vi "Create My API.vi"(5 "My API in":refnum<class "My API.lvclass">, 8 "error in (no error)":errorcluster) -> (0 "error out":errorcluster, 3 "My API out":refnum<class "My API.lvclass">)   [LabVIEW 2017, in "My API.lvclass"]
uses:
  My API.lvclass
  My API.lvclass/My API.ctl
  classes/REST Client/REST Client.lvclass
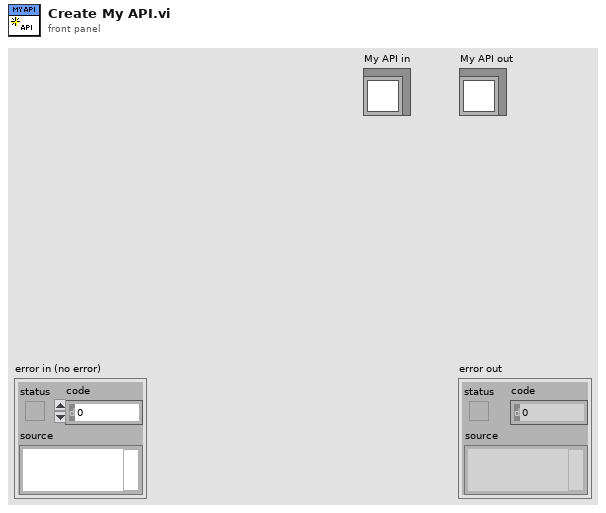
[diagram p1: front panel]
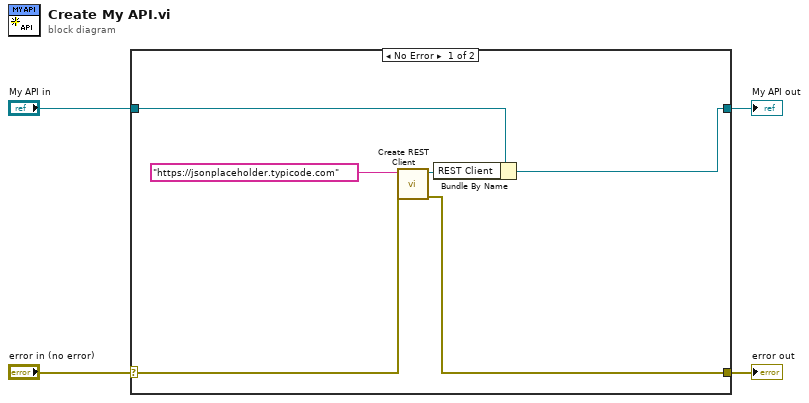
[diagram p0: block diagram]
diagram:
  n1 = case shown="No Error" "error in (no error)" {
    selector: "error in (no error)" -> [w5 w12]
    tunnel: [w6 w12] -> w3
    tunnel: [w7 w11] -> w1
    tunnel: "My API in" -> [w8 w11]
    frame No Error {
      n2 = call "Create REST Client.vi"("error in (no error)"=w5, "Base URL"="https://jsonplaceholder.typicode.com") -> ("error out"=w6:errorcluster, "REST Client out"=w9:refnum<class "REST Client.lvclass">)  [unwired: 8 in]
      n3 = Bundle By Name(cluster=w8, "REST Client"=w9) -> (w7:refnum<class "My API.lvclass">)
    }
    frame Error {
    }
  }
  "error out" <- w3
  "My API out" <- w1
